vi "NR stop Call.vi"(8 "error in (no error)":errorcluster caption="에러 입력(에러 없음)", 11 "Instrument Manager 입력":refnum<class "Instrument Manager.lvclass">) -> (0 "error out":errorcluster caption="에러 출력", 3 "Instrument Manager 출력":refnum<class "Instrument Manager.lvclass">)   [LabVIEW 2023, in "Instrument Manager.lvclass"]
uses:
  Instrument Manager.lvclass
  Instrument Manager.lvclass/Instrument Manager.ctl
  Module/ANRITSU Call Box/Interface Class/Anritsu Call Box.lvclass
  Module/ANRITSU Call Box/Type Definition/Call Processing Command.ctl
  Module/ANRITSU Call Box/ANRITSU Call Box.lvlib
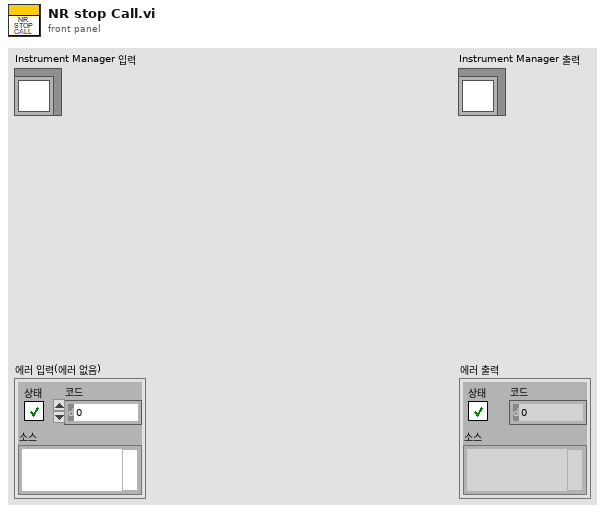
[diagram p1: front panel]
types:
  T1 = typedef "ANRITSU Call Box.lvlib/Call Processing Command.ctl" = enum16{"Start Call", "End Call"}
  T2 = cluster{"Anritsu Call Box":refnum<class "Anritsu Call Box.lvclass">, "Spectrum Analyzer":refnum<class "Interface_Spectrum.lvclass">, "RF Switch Box":refnum<class "RF Filter Box.lvclass">, "Turn Table":refnum<class "Interface - Turn Table.lvclass">, "Mast":refnum<class "Interface - Mast.lvclass">, "3D Controller":refnum<class "Interface_3D Controller.lvclass">}
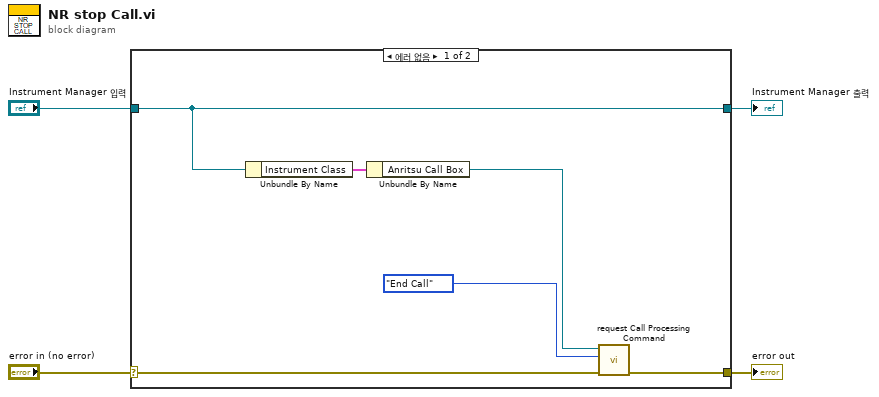
[diagram p0: block diagram]
diagram:
  n1 = case shown="에러 없음" "error in (no error)" {
    selector: "error in (no error)" -> [w7 w12]
    tunnel: [w6 w12] -> w3
    tunnel: [w9 w11] -> w1
    tunnel: "Instrument Manager 입력" -> [w9 w11]
    frame No Error {
      n2 = Unbundle By Name(w9) -> ("Instrument Class"=w10:T2)
      n3 = Unbundle By Name(w10) -> ("Anritsu Call Box"=w8:refnum<class "Anritsu Call Box.lvclass">)
      n4 = call-dynamic "request Call Processing Command.vi"("error in (no error)"=w7, "Call Processing Mode"=Call_Processing_Command."End Call", "Anritsu Call Box in"=w8) -> ("error out"=w6:errorcluster)  [unwired: 7 in, 1 out]
    }
    frame Error {
    }
  }
  "error out" <- w3
  "Instrument Manager 출력" <- w1
